vi "Resource.vi"(8 "error in (no error)":errorcluster, 11 "Channel in":refnum<class "Channel Config.lvclass">) -> (0 "error out":errorcluster, 2 "Resource":string, 3 "Channel out":refnum<class "Channel Config.lvclass">)   [LabVIEW 2020, in "VolatusConfig.lvlib" / "Channel Config.lvclass"]
uses:
  Channel Config.lvclass
  C:/dev/lv20CE/relink/lv-volatus/VolatusConfig/VolatusConfigElement/VolatusConfigElement.lvclass
  VolatusConfigElement/VolatusConfigElement.lvclass/VolatusConfigElement.ctl
  VolatusConfigElement/Element.vi
  Channel Config.lvclass/Channel Config.ctl
  lv-cdm/CDM-Config/Config Element/Config Element.lvclass
  VolatusConfigElement/VolatusConfigElement.lvclass
  C:/dev/lv20CE/relink/lv-volatus/VolatusConfig/Channel/Channel Config.lvclass
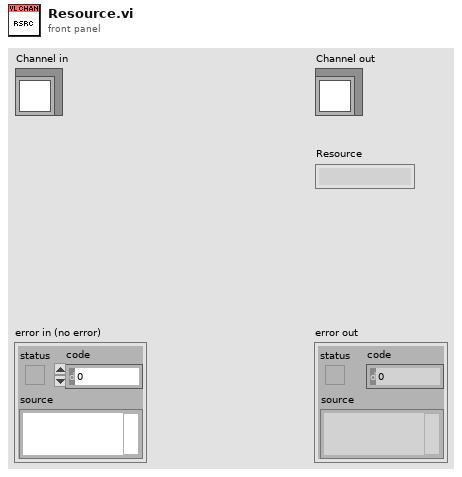
[diagram p1: front panel]
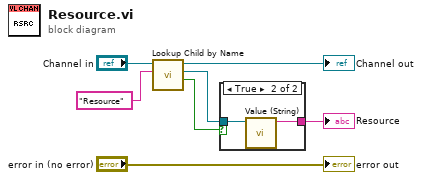
[diagram p0: block diagram]
diagram:
  n1 = call "Lookup Child by Name.vi"("Child Name"="Resource" ("Name"), "VolatusConfigElement in"="Channel in") -> ("Found"=w2:bool, "Child"=w1:refnum<class "Config Element.lvclass">, "VolatusConfigElement out"=→"Channel out":refnum<class "Channel Config.lvclass">)  [unwired: 6 in, 1 out]
  n2 = case shown="True" w2 {
    tunnel: w1 -> [_ w9]
    tunnel: [_ w8] -> w5
    frame False {
    }
    frame True {
      n3 = call "Value (String).vi"("Config Element in"=w9) -> ("String Value"=w8:string)  [unwired: 9 in, 1 out]
    }
  }
  "Resource" <- w5
  "error out" <- "error in (no error)"
